vi "dowhileexample.vi"   [LabVIEW 2015]
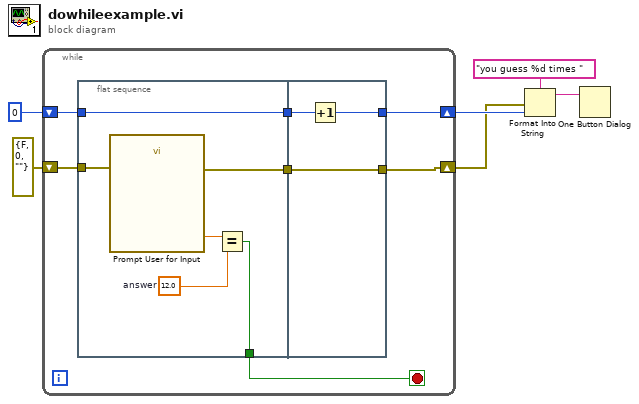
[diagram p0: block diagram]
diagram:
  n1 = while {
    shift-right: [w10] -> w5
    shift-left: 0 -> [w11]
    shift-right: [w8] -> w1
    shift-left: errorcluster {"status"=FALSE, "code"=0, "source"=""} ("error out") -> [w9]
    stop <- w13 stop-if-true
    n2 = flat-sequence {
      tunnel: [w17] -> w13
      tunnel: [w16] -> w12
      tunnel: w11 -> [w16]
      tunnel: w9 -> [w15]
      tunnel: [w14] -> w7
      tunnel: w12 -> [w22]
      tunnel: [w21] -> w10
      tunnel: [w20] -> w8
      tunnel: w7 -> [w20]
      frame #0 {
        w18 = 12.0  # answer
        n3 = call "Prompt User for Input"("error in (no error)"=w15) -> ("your guess?"=w19:dbl, "error out"=w14:errorcluster)  [unwired: 16 in, 1 out]
        n4 = Equal?(x=w19, y=w18) -> (x = y?=w17:bool)
      }
      frame #1 {
        n5 = Increment(x=w22) -> (x+1=w21:i32)
      }
    }
  }
  n6 = Format Into String(format string="you guess %d times ", error in=w1, w5) -> (resulting string=w3:string)  [unwired: 1 in, 1 out]
  n7 = One Button Dialog(message=w3) -> ()  [unwired: 1 in, 1 out]
